vi "Own20261012_SetBooleanStateStrings.vi"() -> ()   [LabVIEW 2024]
panel:
  out "error out":errorcluster caption="错误输出"
  in  "state_strings":string[](array[string])
  in  "boolean_id":u32
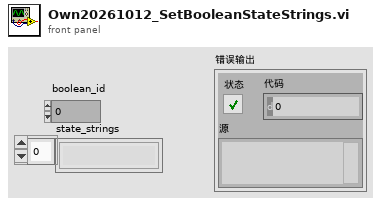
[diagram p1: front panel]
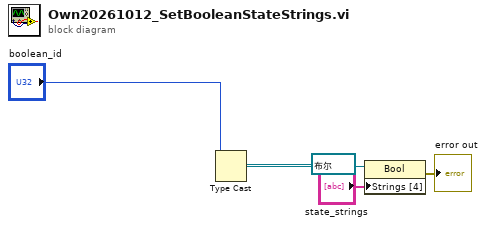
[diagram p0: block diagram]
diagram:
  n1 = Type Cast(type=refnum<vi> refnum ("引用"), x="boolean_id") -> (*(type *) &x=w3:refnum<vi>)
  n2 = property class="Bool"(reference=w3, "Strings [4]"="state_strings") -> (error out=→"error out":errorcluster)  [unwired: 1 in, 1 out]
